vi "ziGetEventPidVector.vi"(8 "Error In":errorcluster, 11 "Handle In":T2 {"Handle" format="0x%08x"; "Conn" format="0x%08x"}) -> (0 "Error Out":errorcluster, 2 "Pid Vector Out":T1, 3 "Handle Out":T2 {"Handle" format="0x%08x"; "Conn" format="0x%08x"})   [LabVIEW 2009, in "Zurich Instruments LabOne.lvlib"]
uses:
  <instrlib>/Zurich Instruments LabOne/Zurich Instruments LabOne.lvlib
  <instrlib>/Zurich Instruments LabOne/Public/ziTypeHandle.ctl
  <instrlib>/Zurich Instruments LabOne/Public/Data/ziTypePidVectorEx.ctl
  <instrlib>/Zurich Instruments LabOne/Private/ziLV64.dll
panel:
  in  "Pid  Vector In":T1
  # "Value"
  # "Value"
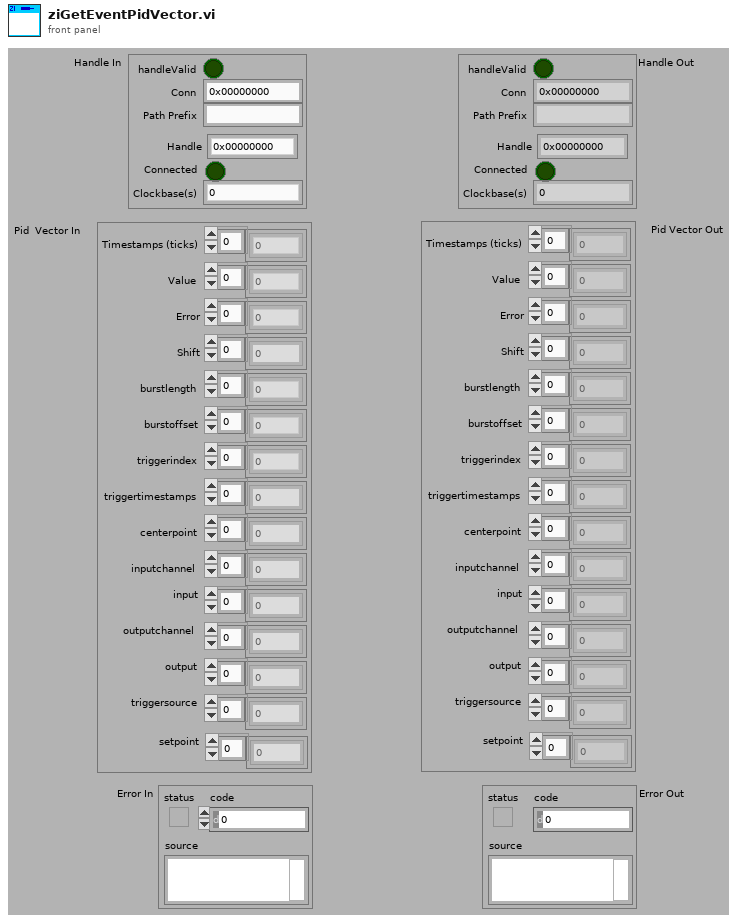
[diagram p1: front panel]
types:
  T1 = typedef "Zurich Instruments LabOne.lvlib/ziTypePidVectorEx.ctl" = cluster{"Timestamps (ticks)":u64[], dbl[], "Error":dbl[], "Shift":dbl[], "burstlength":u32[], "burstoffset":u32[], "triggerindex":u32[], "triggertimestamps":u64[], "centerpoint":dbl[], "inputchannel":u8[], "input":u8[], "outputchannel":u8[], "output":u8[], "triggersource":u8[], "setpoint":dbl[]}
  T2 = typedef "Zurich Instruments LabOne.lvlib/ziTypeHandle.ctl" = cluster{"handleValid":bool, "Conn":u64, "Path Prefix":string, "Handle":u64, "Connected":bool, "Clockbase(s)":dbl}
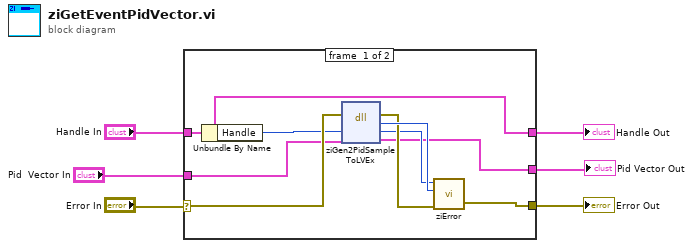
[diagram p0: block diagram]
diagram:
  n1 = case shown="No Error" "Error In" {
    selector: "Error In" -> [w14 w17]
    tunnel: "Handle In" -> [w10 w18]
    tunnel: [w10 w18] -> w5
    tunnel: [w15 w17] -> w4
    tunnel: "Pid  Vector In" -> [w8 w16]
    tunnel: [w7 w16] -> w1
    frame #0 {
      n2 = Unbundle By Name(w10) -> ("Handle"=w13:u64)
      n3 = dll-call lib="C:/Program Files/National Instruments/LabVIEW 2009/instr.lib/Zurich Instruments LabOne/Private/ziLV*.*" fn="ziGen2PidSampleToLVEx"(error in=w14, "ziEventBuffer"=w13, "ShfGhfPidSample"=w8) -> (error out=w11:errorcluster, "return type"=w12:u32, "ziEventBuffer"=w9:u64, "ShfGhfPidSample"=w7:T1)  [unwired: 2 in, 1 out]
      n4 = call <instrlib>:"ziError.vi"("Conn"=w9, "ziErrorCode"=w12, "Error In"=w11) -> ("Error Out"=w15:errorcluster)  [unwired: 2 in, 1 out]
    }
    frame #1 {
    }
  }
  "Handle Out" <- w5
  "Error Out" <- w4
  "Pid Vector Out" <- w1
